vi "Recuperation donnees precedentes.vi"() -> (2 "Données":dbl[][](array[numeric]), 3 "Temps":dbl[](array[numeric]), 4 "commentaire":string, 5 "offset (en octets)":i64)   [LabVIEW 2022 SP3]
uses:
  Variables globales/Variable glob generale.vi
panel:
  out "tableau":string[][](array[string])
  out "Chemin du fichier local :":path
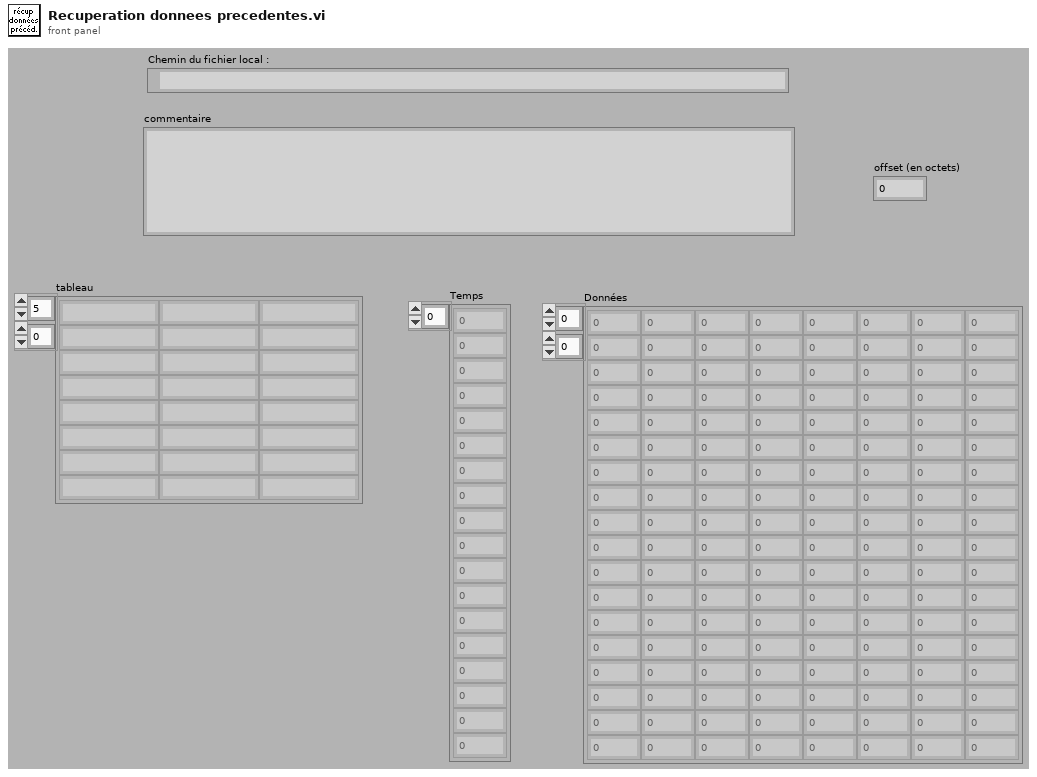
[diagram p1: front panel]
types:
  T1 = enum16{"open", "replace", "create", "open or create", "replace or create", "replace or create with confirmation"}
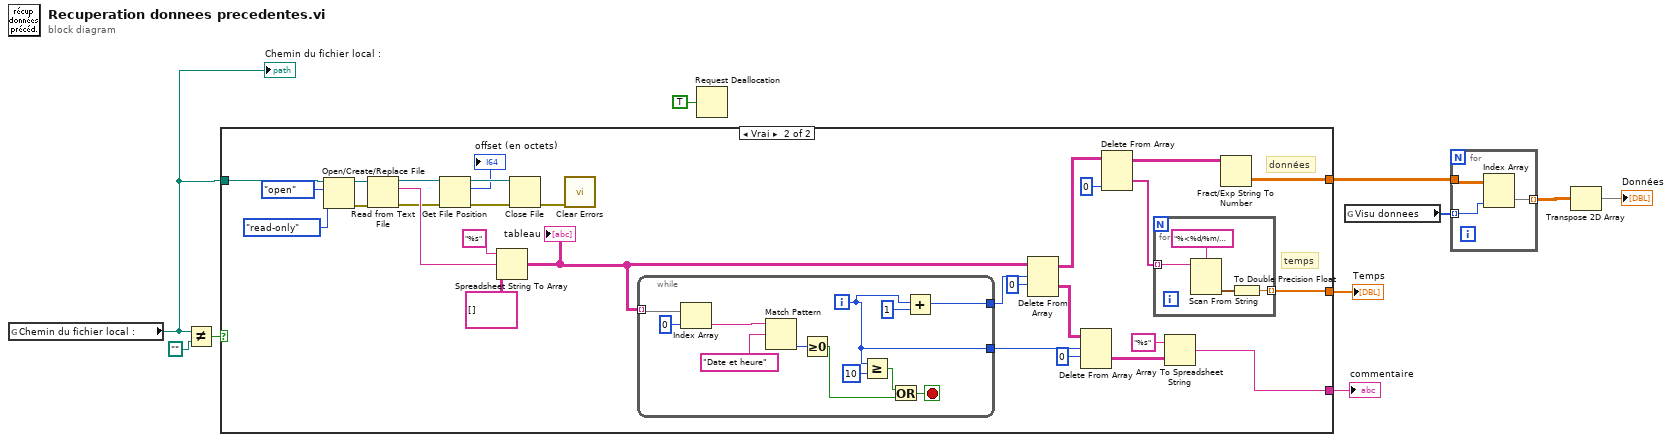
[diagram p0: block diagram]
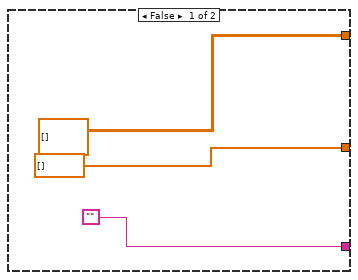
[diagram p2: hidden frame]
diagram:
  n1 = global read "Variable glob generale.vi" "Chemin du fichier local :"() -> (w1:path)
  "Chemin du fichier local :" <- w1
  n2 = Not Equal?(x=w1, y=path "") -> (x != y?=w10:bool)
  n3 = case shown="Vrai" w10 {
    tunnel: [dbl[][] [] w20] -> w4
    tunnel: [dbl[] [] w17] -> w8
    tunnel: ["" w14] -> w7
    tunnel: w1 -> [_ w30]
    frame False {
    }
    frame True {
      # "données"
      # "temps"
      n4 = Open/Create/Replace File(file path (use dialog)=w30, operation (0:open)=T1."open" ("opération (0 : open)"), access (0:read/write)=enum16{"read/write", "read-only", "write-only"}."read-only" ("accès (0 : read/write)")) -> (refnum out=w29:refnum<file>, error out=w25:errorcluster)  [unwired: 3 in, 1 out]
      n5 = Read from Text File(file (use dialog)=w29, error in=w25) -> (refnum out=w28:refnum<file>, text=w33:string, error out=w24:errorcluster)  [unwired: 2 in, 1 out]
      n6 = Get File Position(4:w24, 7:w28) -> (0:w23:errorcluster, 2:→"offset (en octets)":i64, 3:w27:refnum<file>)
      n7 = Spreadsheet String To Array(format string="%s" ("chaîne de format"), spreadsheet string=w33, array type (2D Dbl)=string[][] [] ("type de tableau (2D de dbl)")) -> (array=w39:string[][])  [unwired: 1 in]
      "tableau" <- w39
      n8 = Close File(refnum=w27, error in=w23) -> (error out=w22:errorcluster)  [unwired: 1 out]
      n9 = call <vilib>:"Clear Errors.vi"("error in (no error)"=w22) -> ()  [unwired: 5 in, 2 out]
      n10 = while {
        tunnel: w39 -> [w58] mode=indexing
        tunnel: [w48] -> w38
        tunnel: [w49] -> w35
        i -> [w49]
        stop <- w54 stop-if-true
        n11 = Index Array(array=w58, index=0 ("indice")) -> (element=w53:string)
        n12 = Match Pattern(string=w53, regular expression="Date et heure") -> (offset past match=w51:i32)  [unwired: 1 in, 3 out]
        n13 = Greater Or Equal To 0?(x=w51) -> (x >= 0?=w50:bool)
        n14 = Greater Or Equal?(x=w49, y=10) -> (x >= y?=w55:bool)
        n15 = Or(x=w55, y=w50) -> (x .or. y?=w54:bool)
        n16 = Add(x=w49, y=1) -> (x+y=w48:i32)
      }
      n17 = Delete From Array(array=w39, length=w38, index (row)=0 ("indice (ligne)")) -> (deleted portion=w36:string[][], array with subset deleted=w19:string[][])  [unwired: 1 in]
      n18 = Delete From Array(array=w36, length=w35, index (row)=0 ("indice désactivé (col)")) -> (deleted portion=w16:string[][])  [unwired: 1 in, 1 out]
      n19 = Delete From Array(array=w19, index (col)=0 ("indice désactivé (col)")) -> (deleted portion=w18:string[], array with subset deleted=w21:string[][])  [unwired: 2 in]
      n20 = for {
        tunnel: w18 -> [w44] mode=indexing
        tunnel: [w43] -> w17 mode=indexing
        n21 = Scan From String(format string="%<%d/%m/%Y%2u%H:%M:%S>T" ("chaîne de format"), input string=w44) -> (output 1=w45:timestamp)  [unwired: 3 in, 3 out]
        n22 = To Double Precision Float(number=w45) -> (double precision float=w43:dbl)
      }
      n23 = Array To Spreadsheet String(array=w16, 3:"%s" ("chaîne de format")) -> (spreadsheet string=w14:string)  [unwired: 1 in]
      n24 = Fract/Exp String To Number(string=w21) -> (number=w20:dbl[][])  [unwired: 3 in, 1 out]
    }
  }
  "Temps" <- w8
  "commentaire" <- w7
  n25 = Request Deallocation(TRUE ("flag")) -> ()
  n26 = global read "Variable glob generale.vi" "Visu donnees"() -> (w5:i32[])
  n27 = for {
    tunnel: w5 -> [w60] mode=indexing
    tunnel: w4 -> [w61]
    tunnel: [w59] -> w3 mode=indexing
    n28 = Index Array(array=w61, index (col)=w60) -> (element=w59:dbl[])  [unwired: 1 in]
  }
  n29 = Transpose 2D Array(2D array=w3) -> (transposed array=→"Données":dbl[][])
